vi "GDSString_ParseDataTypeString.vi"(6 "Classes":T1[](array[typedef]), 10 "DefaultAccessScope(Private)":T2, 11 "InputText":string) -> (1 "DataTypeString":string, 2 "Found":bool, 3 "DataType":T3)   [LabVIEW 2020]
uses:
  CommonVIs/CommonVIs_AttributeType.ctl
  CommonVIs/CommonVIs_AttributeDataType.ctl
  GDSString_AccessScopeModifierType.ctl
  CommonVIs/CommonVIs_ClassNamePathType.ctl
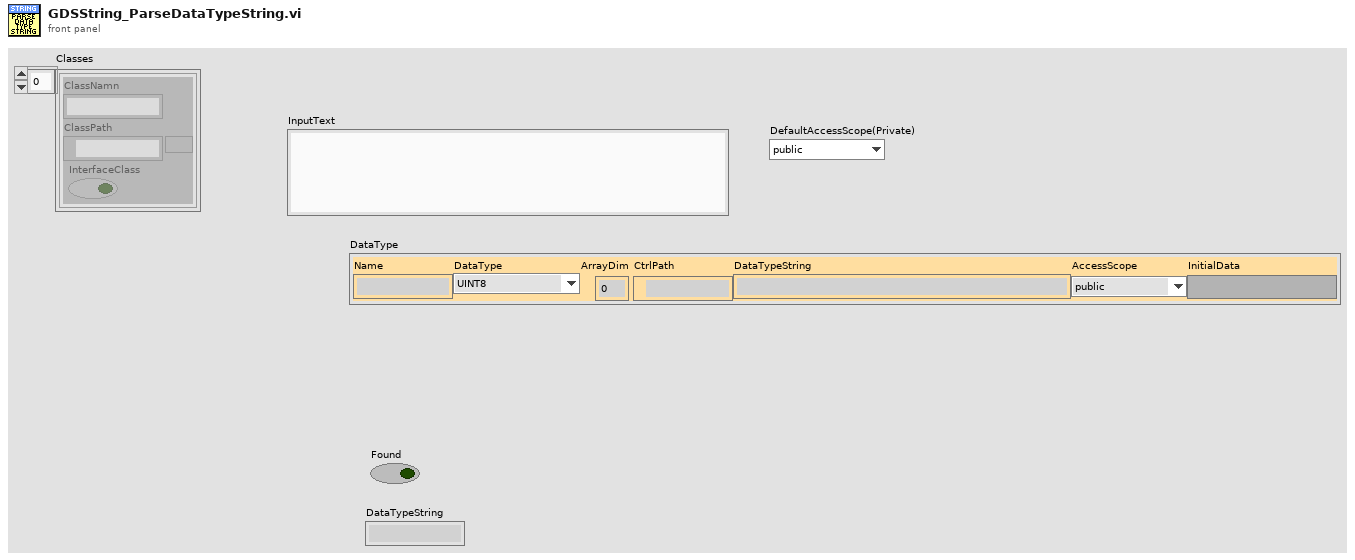
[diagram p1: front panel]
types:
  T1 = typedef "CommonVIs_ClassNamePathType.ctl" = cluster{"ClassNamn":string, "ClassPath":path, "InterfaceClass":bool}
  T2 = typedef "GDSString_AccessScopeModifierType.ctl" = enum16{"public", "private", "protected", "internal"}
  T3 = typedef "CommonVIs_AttributeType.ctl" = cluster{"Name":string, "DataType":T4, "ArrayDim":i32, "CtrlPath":path, "DataTypeString":string, "AccessScope":T2, "InitialData":variant}
  T4 = typedef "CommonVIs_AttributeDataType.ctl" = enum16{"UINT8", "INT8", "UINT16", "INT16", "UINT32", "INT32", "UINT64", "INT64", "SGL", "DBL", "EXT", "CSG", "CDB", "CXT", "TimeStamp", "STRING", "PATH", "BOOL", "ENUM", "RefNum", "VIRefNum", "LabVIEW Class", "Cluster", "Variant", "TypeDef", "Waveform", "LabVIEW Object", "Other", "void", "Set", "Map"}
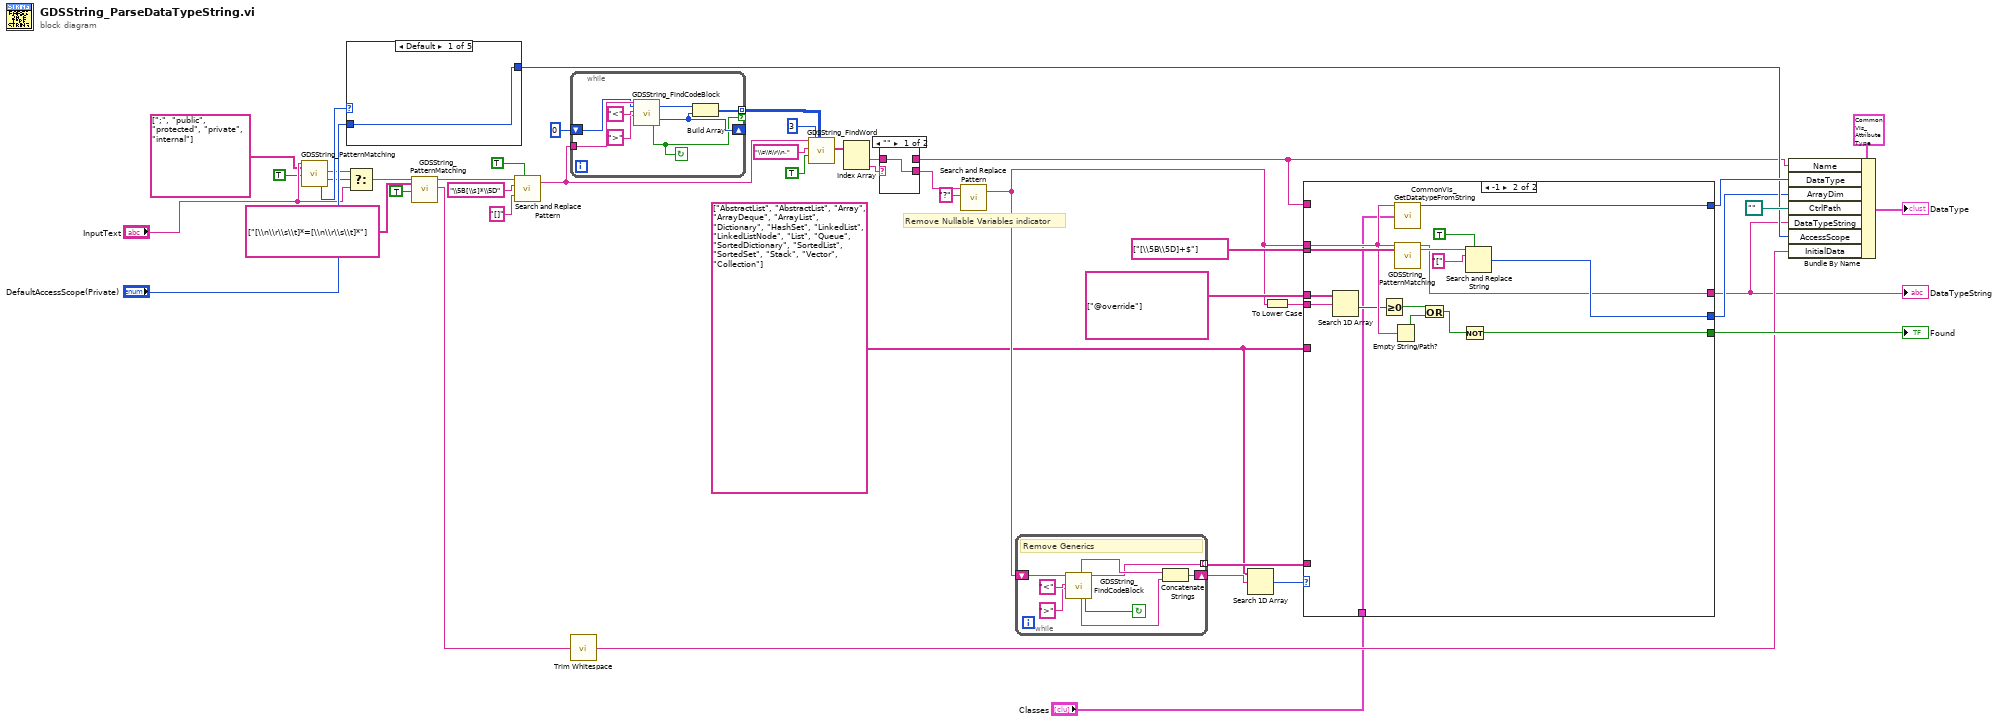
[diagram p0: block diagram]
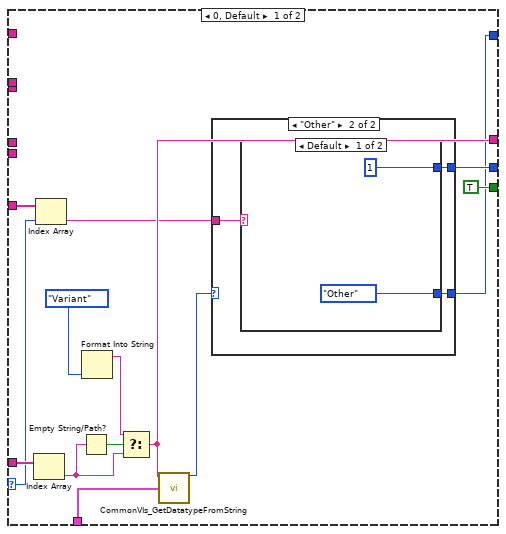
[diagram p3: hidden frame]
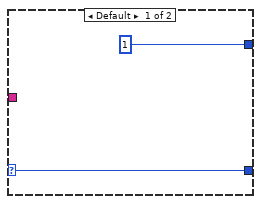
[diagram p4: hidden frame]
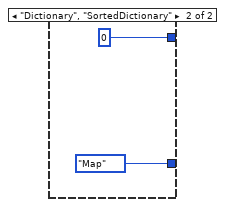
[diagram p5: hidden frame]
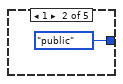
[diagram p6: hidden frame]
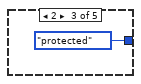
[diagram p7: hidden frame]
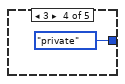
[diagram p8: hidden frame]
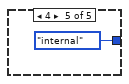
[diagram p9: hidden frame]
diagram:
  w2 = string[] ["AbstractList", "AbstractList", "Array", "ArrayDeque", "ArrayList", "Dictionary", "HashSet", "LinkedList", "LinkedListNode", "List", "Queue", "SortedDictionary", "SortedList", "SortedSet", "Stack", "Vector", "Collection"] ("array")
  # "Remove Nullable Variables indicator"
  n1 = call "GDSString_PatternMatching.vi"("TextIn"="InputText", "PatternMatchingStrings"=string[] [";", "public", "protected", "private", "internal"] ("PatternMatchingString"), "Search Backwards"=TRUE) -> ("IndexOfTheFoundPatternMatchingString"=w31:i32, "TextAfter"=w24:string, "Found"=w23:bool)  [unwired: 10 in, 4 out]
  n2 = case shown="Default" w31 {
    tunnel: [w46 GDSString_AccessScopeModifierType."public" ("AccessScope") GDSString_AccessScopeModifierType."protected" ("AccessScope") GDSString_AccessScopeModifierType."private" ("AccessScope") GDSString_AccessScopeModifierType."internal" ("AccessScope")] -> w34
    tunnel: "DefaultAccessScope(Private)" -> [w46 _ _ _ _]
    frame Default {
    }
    frame 1 {
    }
    frame 2 {
    }
    frame 3 {
    }
    frame 4 {
    }
  }
  n3 = Select(t=w24, s=w23, f="InputText") -> (s? t:f=w26:string)
  n4 = call "GDSString_PatternMatching.vi"("TextIn"=w26, "PatternMatchingStrings"=string[] ["[\\n\\r\\s\\t]*=[\\n\\r\\s\\t]*"] ("PatternMatchingString"), "Search Backwards"=TRUE) -> ("TextBefore"=w38:string, "TextAfter"=w35:string)  [unwired: 10 in, 5 out]
  n5 = call <vilib>:"Search and Replace Pattern.vi"("string"=w38, "regular expression (\"\")"="\\5B[\\s]*\\5D" ("regular expression (\"\")"), "replace string (\"\")"="[]" ("replace string (\"\")"), "replace all? (F)"=TRUE) -> ("result string"=w11:string)  [unwired: 1 in, 1 out]
  n6 = while {
    tunnel: w11 -> [w58]
    shift-right: [w57] -> _
    shift-left: 0 ("offset past match") -> [w56]
    tunnel: [w55] -> w10 mode=indexing if=w54
    stop <- w54 continue-if-true
    n7 = call "GDSString_FindCodeBlock.vi"("Text"=w58, "StringStartOffset(Default=-1 => 0 for Forward, StrLenght for Backwards)"=w56, "CodeBlockStartCharacter( { )"="<", "CodeBlockEndCharacter( } )"=">") -> ("found"=w54:bool, "BlockStart(Outside)"=w51:i32, "BlockEnd(Outside)"=w57:i32)  [unwired: 7 in, 6 out]
    n8 = Build Array(w51, w57) -> (w55:i32[])
  }
  n9 = call <vilib>:"Trim Whitespace.vi"("string"=w35) -> ("trimmed string"=w36:string)  [unwired: 1 in]
  n10 = call "GDSString_FindWord.vi"("Text"=w11, "PatternMatchingDelimiter(\\s\\t\\r\\n)"="\\s\\t\\r\\n," ("PatternMatchingDelimiter(\\s\\t\\r\\n)"), "Search Backwards"=TRUE, "GetNext-X_Words(1,-1=All)"=3, "IgnoreMatchesWithinThesePositions"=w10) -> ("NextWords"=w14:string[])  [unwired: 9 in, 5 out]
  n11 = Index Array(array=w14) -> (element #1=w20:string, element #2=w13:string)  [unwired: 2 in]
  n12 = case shown="\"\"" w13 {
    selector: w13 -> [_ w60]
    tunnel: w20 -> [w59 w61]
    tunnel: [_ w61] -> w19
    tunnel: [w59 w60] -> w5
    frame "" {
    }
    frame Default {
    }
  }
  n13 = call <vilib>:"Search and Replace Pattern.vi"("string"=w5, "regular expression (\"\")"="?" ("regular expression (\"\")")) -> ("result string"=w4:string)  [unwired: 3 in, 1 out]
  n14 = while {
    shift-right: [w63] -> w16
    shift-left: w4 -> [w69]
    tunnel: [w62] -> w15 mode=indexing
    stop <- w66 continue-if-true
    # "Remove Generics"
    n15 = call "GDSString_FindCodeBlock.vi"("Text"=w69, "CodeBlockStartCharacter( { )"="<", "CodeBlockEndCharacter( } )"=">") -> ("TextBeforeBlock"=w65:string, "TextAfterBlock"=w64:string, "found"=w66:bool, "BlockText"=w62:string)  [unwired: 8 in, 5 out]
    n16 = Concatenate Strings(w65, w64) -> (w63:string)
  }
  n17 = Search 1D Array(1D array=w2, element=w16) -> (index of element=w17:i32)  [unwired: 1 in]
  n18 = To Lower Case(string=w4) -> (all lower case string=w7:string)
  n19 = case shown="-1" w17 {
    selector: w17 -> [w72 _]
    tunnel: [w74 w108] -> w45
    tunnel: [TRUE w102] -> w43
    tunnel: [w76 w106] -> w33
    tunnel: string[] ["[\\5B\\5D]+$"] ("PatternMatchingString") -> [_ w103]
    tunnel: w19 -> [_ _]
    tunnel: w4 -> [_ w101]
    tunnel: w15 -> [w82 _]
    tunnel: [w80 w100] -> w9
    tunnel: string[] ["@override"] ("PatternMatchingString") -> [_ w99]
    tunnel: w7 -> [_ w98]
    tunnel: w2 -> [w73 _]
    tunnel: "Classes" -> [w70 w93]
    frame 0, Default {
      n20 = Index Array(array=w82) -> (element=w79:string)  [unwired: 1 in]
      n21 = Index Array(array=w73, index=w72) -> (element=w71:string)
      n22 = Empty String/Path?(string/path=w79) -> (empty?=w81:bool)
      n23 = Format Into String(CommonVIs_AttributeDataType."Variant" ("DataType")) -> (resulting string=w77:string)  [unwired: 3 in, 1 out]
      n24 = Select(t=w77, s=w81, f=w79) -> (s? t:f=w80:string)
      n25 = call "CommonVIs_GetDatatypeFromString.vi"("String"=w80, "Classes"=w70) -> ("AttributeDataType"=w75:T4)  [unwired: 9 in, 4 out]
      n26 = case shown="\"Other\"" w75 {
        selector: w75 -> [w84 _]
        tunnel: [1 ("number of replacements") w88] -> w76
        tunnel: [w84 w87] -> w74
        tunnel: w71 -> [_ w86]
        frame Default {
        }
        frame "Other" {
          n27 = case shown="Default" w86 {
            tunnel: [1 ("number of replacements") 0 ("number of replacements")] -> w88
            tunnel: [CommonVIs_AttributeDataType."Other" ("AttributeDataType") CommonVIs_AttributeDataType."Map" ("AttributeDataType")] -> w87
            frame Default {
            }
            frame "Dictionary", "SortedDictionary" {
            }
          }
        }
      }
    }
    frame -1 {
      n28 = Search 1D Array(1D array=w99, element=w98) -> (index of element=w97:i32)  [unwired: 1 in]
      n29 = Greater Or Equal To 0?(x=w97) -> (x >= 0?=w96:bool)
      n30 = Empty String/Path?(string/path=w101) -> (empty?=w95:bool)
      n31 = call "CommonVIs_GetDatatypeFromString.vi"("String"=w101, "Classes"=w93) -> ("AttributeDataType"=w108:T4)  [unwired: 9 in, 4 out]
      n32 = call "GDSString_PatternMatching.vi"("TextIn"=w101, "PatternMatchingStrings"=w103) -> ("TextBefore"=w100:string, "Match"=w104:string)  [unwired: 11 in, 5 out]
      n33 = Or(x=w96, y=w95) -> (x .or. y?=w94:bool)
      n34 = Not(x=w94) -> (.not. x?=w102:bool)
      n35 = Search and Replace String(replace all?=TRUE ("replace all? (F)"), input string=w104, search string="[") -> (number of replacements=w106:i32)  [unwired: 5 in, 3 out]
    }
  }
  "Found" <- w43
  "DataTypeString" <- w9
  n36 = Bundle By Name(cluster=T3 {"Name"="", "DataType"=enum."UINT8", "ArrayDim"=0, "CtrlPath"=path "", "DataTypeString"="", "AccessScope"=enum."public", "InitialData"=variant} ("DataType"), "Name"=w19, "DataType"=w45, "ArrayDim"=w33, "CtrlPath"=path "", "DataTypeString"=w9, "AccessScope"=w34, "InitialData"=w36) -> (→"DataType":T3)
